vi "create run.vi"(9 "Start Time (now)":timestamp format="%<%x %.3X>T", 10 "Title":string, 11 "connection":refnum<class "Nominal Client.lvclass">) -> (0 "error out":errorcluster, 3 "Run":refnum<class "Run.lvclass">)   [LabVIEW 2020, in "nominal core steps.lvlib"]
doc: "Creates a run without an associated asset. Runs have a start and end time, with start time required."
uses:
  nominal core steps.lvlib
  <vilib>/Nominal/Nominal IO Client/lv_src/Nominal Client/Nominal Client.lvclass
  <vilib>/Nominal/Nominal IO Client/lv_src/Run/Run.lvclass
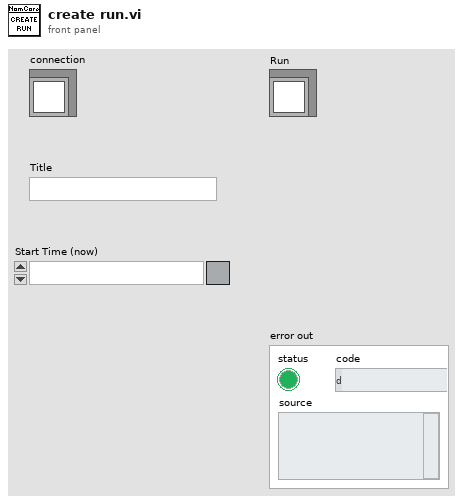
[diagram p1: front panel]
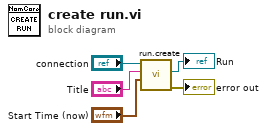
[diagram p0: block diagram]
diagram:
  n1 = call <vilib>:"run.create.vi"("Start Time (now)"="Start Time (now)", "Title"="Title", "Nominal Client in"="connection") -> ("error out"=→"error out":errorcluster, "Run"=→"Run":refnum<class "Run.lvclass">)  [unwired: 6 in, 1 out]
